vi "NEO Get Sensor Values.vi"(11 "Motors In":T1 {"Steer Scaling" format="%.2f"; "Drive Scaling" format="%.2f"; "Pod Locations (ft)"."Right Back Position" format="%.2f"; "Pod Locations (ft)"."Right Front Position" format="%.2f"; "Pod Locations (ft)"."Left Back Position" format="%.2f"; "Pod Locations (ft)"."Left Front Position" format="%.2f"}) -> (2 "Steer Angles (degrees)":T4, 3 "Drive Velocities (ft/s)":T4)   [LabVIEW 2027]
uses:
  Type Definitions/Hardware/Swerve Drives/(NEO-NEO-ThroughBore-Pigeon2) Swerve.ctl
  <vilib>/REV Custom Controls/REVSparkRefnum.ctl
  Type Definitions/Data/Pod Positions.ctl
  <resource>/objmgr/REVSpark.rc
  <vilib>/REVLibDriver/REVLibDriver.lvlib
panel:
  in  "Max Delay":u32
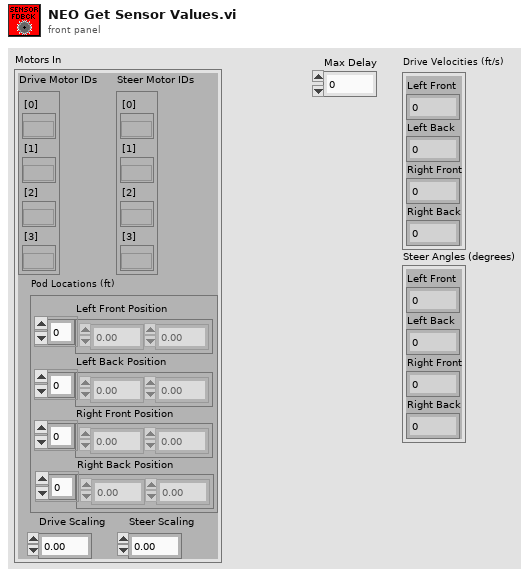
[diagram p1: front panel]
types:
  T1 = typedef "(NEO-NEO-ThroughBore-Pigeon2) Swerve.ctl" = cluster{"Drive Motor IDs":cluster{"[0]":T2, "[1]":T2, "[2]":T2, "[3]":T2}, "Steer Motor IDs":cluster{"[0]":T2, "[1]":T2, "[2]":T2, "[3]":T2}, "Pod Locations (ft)":T3, "Drive Scaling":dbl, "Steer Scaling":dbl}
  T2 = typedef "REVLibDriver.lvlib/REVSparkRefnum.ctl" = refnum<k20>
  T3 = typedef "Pod Positions.ctl" = cluster{"Left Front Position":dbl[], "Left Back Position":dbl[], "Right Front Position":dbl[], "Right Back Position":dbl[]}
  T4 = cluster{"Left Front":dbl, "Left Back":dbl, "Right Front":dbl, "Right Back":dbl}
  T5 = cluster{"[0]":dbl, "[1]":dbl, "[2]":dbl, "[3]":dbl}
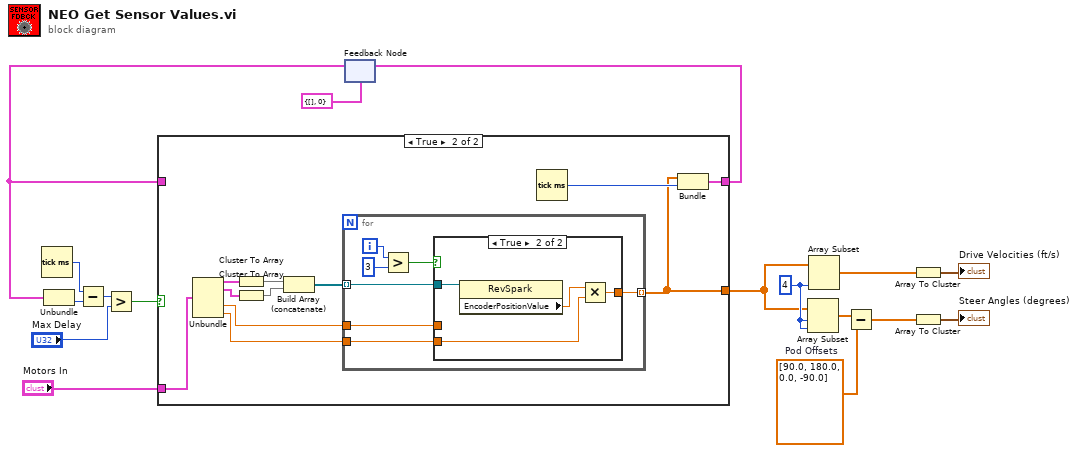
[diagram p0: block diagram]
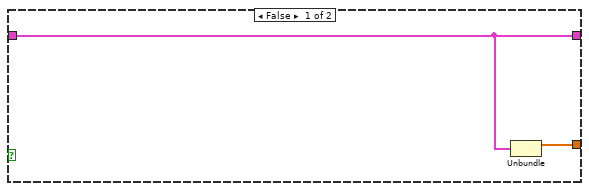
[diagram p2: hidden frame]
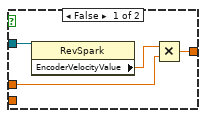
[diagram p3: hidden frame]
diagram:
  w12 = dbl[] [90.0, 180.0, 0.0, -90.0]  # Pod Offsets
  w16 = 4 ("length")
  n1 = Tick Count (ms)() -> (millisecond timer value=w8:u32)
  n2 = feedback #1(cluster{dbl[], "millisecond timer value":u32} {[], "millisecond timer value"=0}) -> (w7:cluster{dbl[], "millisecond timer value":u32})
  n3 = Unbundle(w7) -> ("millisecond timer value"=w6:u32)  [unwired: 1 out]
  n4 = Subtract(x=w8, y=w6) -> (x-y=w5:u32)
  n5 = Greater?(x=w5, y="Max Delay") -> (0:w3:bool)
  n6 = case shown="True" w3 {
    tunnel: [w18 w24] -> w10
    tunnel: [w19 w23] -> w9
    tunnel: w7 -> [w19 _]
    tunnel: "Motors In" -> [_ w22]
    frame False {
      n7 = Unbundle(w19) -> (w18:dbl[])  [unwired: 1 out]
    }
    frame True {
      n8 = Unbundle(w22) -> ("Drive Motor IDs"=w30:cluster{"[0]":T2, "[1]":T2, "[2]":T2, "[3]":T2}, "Steer Motor IDs"=w29:cluster{"[0]":T2, "[1]":T2, "[2]":T2, "[3]":T2}, "Drive Scaling"=w21:dbl, "Steer Scaling"=w20:dbl)  [unwired: 1 out]
      n9 = Cluster To Array(cluster=w30) -> (array=w28:T2[])
      n10 = Cluster To Array(cluster=w29) -> (array=w27:T2[])
      n11 = Build Array (concatenate)(w28, w27) -> (w26:T2[])
      n12 = for {
        tunnel: w26 -> [w35] mode=indexing
        tunnel: [w34] -> w24 mode=indexing
        tunnel: w21 -> [w32]
        tunnel: w20 -> [w31]
        i -> [w36]
        n13 = Greater?(x=w36, y=3) -> (0:w33:bool)
        n14 = case shown="True" w33 {
          tunnel: w35 -> [w41 w45]
          tunnel: [w40 w44] -> w34
          tunnel: w32 -> [w38 _]
          tunnel: w31 -> [_ w42]
          frame False {
            n15 = property class="RevSpark"(reference=w41) -> ("EncoderVelocityValue"=w39:sgl)  [unwired: 1 in, 2 out]
            n16 = Multiply(x=w39, y=w38) -> (x*y=w40:dbl)
          }
          frame True {
            n17 = property class="RevSpark"(reference=w45) -> ("EncoderPositionValue"=w43:sgl)  [unwired: 1 in, 2 out]
            n18 = Multiply(x=w43, y=w42) -> (x*y=w44:dbl)
          }
        }
      }
      n19 = Tick Count (ms)() -> (millisecond timer value=w25:u32)
      n20 = Bundle(w24, "millisecond timer value"=w25) -> (w23:cluster{dbl[], "millisecond timer value":u32})  [unwired: 1 in]
    }
  }
  n21 = feedback-in #1(w9) -> ()
  n22 = Array Subset(array=w10, index=w16, length=w16) -> (w13:dbl[])
  n23 = Array Subset(array=w10, length=w16) -> (w17:dbl[])  [unwired: 1 in]
  n24 = Subtract(x=w13, y=w12) -> (x-y=w11:dbl[])
  n25 = Array To Cluster(array=w17) -> (cluster=→"Drive Velocities (ft/s)":T5)
  n26 = Array To Cluster(array=w11) -> (cluster=→"Steer Angles (degrees)":T5)
